vi "VIH Dialog - Project File Rules.vi"(6 "File set (All)":enum32{"ALL", "lost"}(ring), 11 "Project Tree":T1) -> (0 "OK out":bool, 2 "File Paths":path[](array[path]))   [LabVIEW 2014]
doc: "::: VI Helpeks :::\nCopyright (c) 2000-2026 Konstantin Shifershteyn. All rights reserved."
uses:
  VIH Project Tree Typedef - Tree Refnum.ctl
  _VIH HelpGen - Palette.llb/VIH HelpGen Typedef - Palette - Item Type Enum.ctl
  <vilib>/Utility/miscctls.llb/LVRowAndColumnUnsignedTypeDef.ctl
panel:
  in  "QualifiedNames":bool caption="Show qualified VI names"
  in  "KindOfFile":enum16{"All File Rules", "Lost Rules"}(ring) caption="Category Selector"
  in  "DirectSortColumn":i32
  in  "Files tmp":path[](array[path])
  in  "FileList":i32[](listbox) caption="Rule List"
  in  "%OK":bool
  out "Sel Path":path caption="File Path"
  in  "%Cancel":bool caption="Cloce"
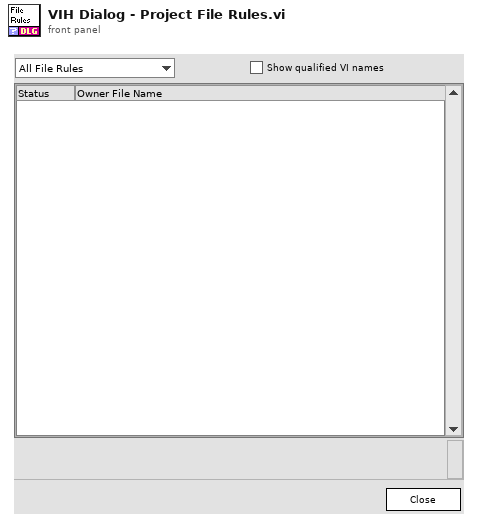
[diagram p1: front panel]
types:
  T1 = typedef "VIH Project Tree Typedef - Tree Refnum.ctl" = refnum<vi>
  T2 = typedef "VIH HelpGen Typedef - Palette - Item Type Enum.ctl" = enum32{"<Invalid>", "<unknown>", "VI", "Menu", "LV Func", "Express VI", "Poly VI", "CTL", "HTML"}
  T3 = cluster{"Types":T2[], "Item Paths":path[], "Lost Flags":bool[], "Names":string[]}
  T4 = enum8{"Enabled", "Disabled", "Disabled and Grayed Out"}
  T5 = enum16{"get", "get all", "set", "Init", "delete", "rename"}
  T6 = typedef "LVRowAndColumnUnsignedTypeDef.ctl" = cluster{"Row":u32, "Column":u32}
  T7 = typedef "LVPoint32TypeDef.ctl" = cluster{"Horizontal":i32, "Vertical":i32}
  T8 = typedef "LVRowAndColumnTypeDef.ctl" = cluster{"Row":i32, "Column":i32}
  T9 = typedef "lveventtype.ctl" = enum32{"Null", "Timeout", "Annotation Menu Selection", "Annotation Menu Selection?", "App Instance Close", "App Instance Close?", "Autoscale Range Change", "Bookmark Info Change", "Cell Edit", "Cell Edit?", "Cursor Grab", "Cursor Grab?", "Cursor Menu Selection", "Cursor Menu Selection?", "Cursor Move", "Cursor Release", "Data Change", "Direction Change", "Display State Change", "Drag Ended", "Drag Enter", "Drag Leave", "Drag Over", "Drag Source Update", "Drag Starting", "Drag Starting?", "Drop", "Exec State Change", "Key Down", "Key Down?", "Key Repeat", "Key Repeat?", "Key Up", "Listbox Double Click", "Menu Activation?", "Menu Selection (App)", "Menu Selection? (App)", "Menu Selection (User)", "Mouse Down", "Mouse Down?", "Mouse Enter", "Mouse Leave", "Mouse Move", "Mouse Up", "Mouse Wheel", "NI Security User Change (App)", "Pane Size", "Panel Close", "Panel Close?", "Panel Resize", "Plot Attribute Change", "Scale Range Change", "Shortcut Menu Activation?", "Shortcut Menu Selection (App)", "Shortcut Menu Selection? (App)", "Shortcut Menu Selection (User)", "Tree Double Click", "Tree Drag", "Tree Drag?", "Tree Drop", "Tree Drop?", "Tree Item Close", "Tree Item Close?", "Tree Item Open", "Tree Item Open?", "User Event", "Value Change"}
  T10 = cluster{"Item/File Type":T2, "Item ID out":path, bool}
  T11 = cluster{"Types":T2[], "Paths":path[], "Dynamic":enum16{"Dyn", "Stat", "Both"}[], "Can be built":bool[], "DynFileNotFound":bool[]}
  T12 = cluster{T2[], "Item Paths":path[], bool[], string[]}
  T13 = typedef "VIH HelpGen Typedef - Cluster - File Rule.ctl" = cluster{"OutName":string, "BuildHelp":T14, "Source Paths":T15, "Target Paths":T16, "DscrMode":T17, "Description":string, "Control Rules":T18[], "Flags":T20, "Ctl_DscrMode":T17, "Ctl_ClustMembers":T14, "Ctl_EnumValues":T14, "MenuItemIcons":T14, "%Comments":string, "DetailsMode":T17, "DetailsText":string, "ProductInfoMode":T14, "ProductInfoText":string}
  T14 = typedef "VIH HelpGen Typedef - Enum - Default,Enable,Disable.ctl" = enum16{"Default", "Enable", "Disable"}
  T15 = typedef "VIH HelpGen Typedef - Cluster - File Rule - Source Paths.ctl" = cluster{"CSS Files":path[], "JS Files":path[], "Html Template":path}
  T16 = typedef "VIH HelpGen Typedef - Cluster - File Rule - Target Paths.ctl" = cluster{"HTML Dir":path, "Image Dir":path, "CSS Dir":path, "JS Dir":path}
  T17 = typedef "VIH HelpGen Typedef - Enum - Description Mode.ctl" = enum16{"Default", "Description", "Description1", "Description2", "Custom", "None"}
  T18 = typedef "VIH HelpGen Typedef - Cluster - Control Rule.ctl" = cluster{"CtrlID":string, "CustomRule":bool, "DscrMode":T17, "Description":string, "ClusterMembers":T14, "EnumValues":T14, "EnumValDscr":T19[], "CustomName":string}
  T19 = typedef "VIH HelpGen Typedef - Cluster - Enum Value Info.ctl" = cluster{"Value":ext, "String":string, "Description":string}
  T20 = typedef "VIH HelpGen Typedef - Cluster - Group Rule - Flags.ctl" = cluster{"Override CSS Files":bool, "Override JS Files":bool, "Override Ctl Rules":bool}
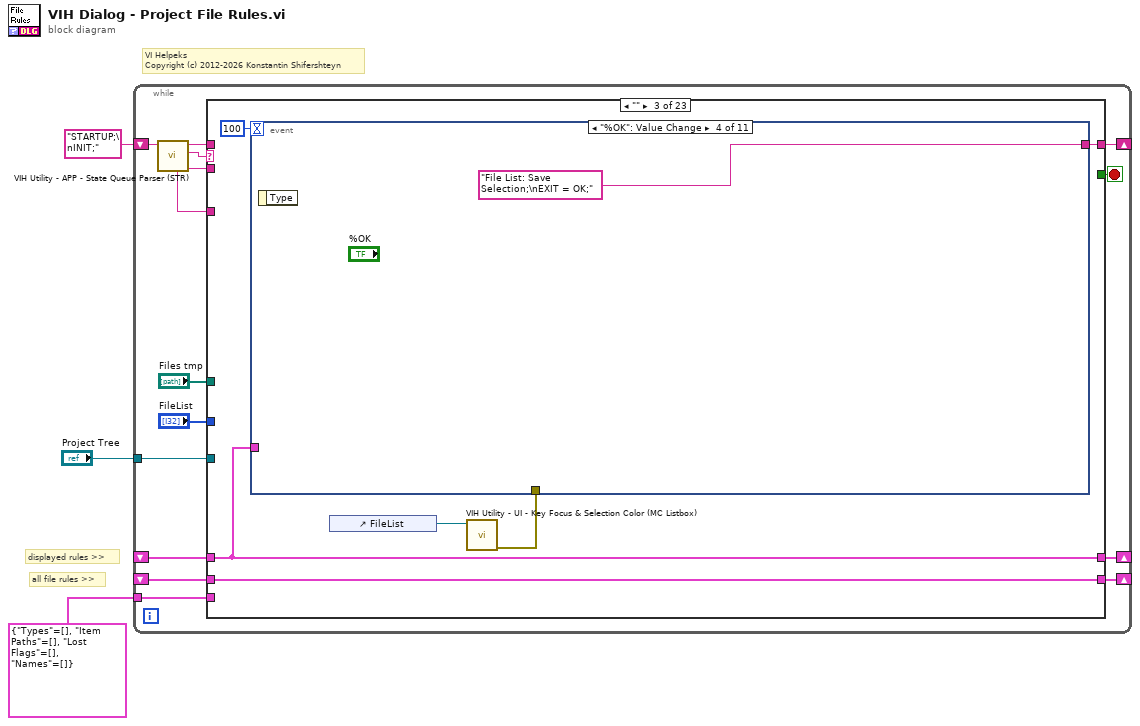
[diagram p0: block diagram]
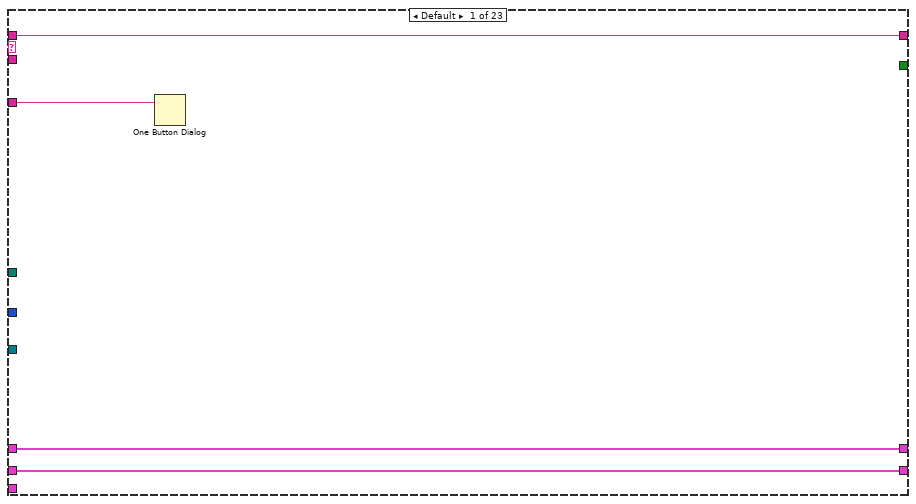
[diagram p2: hidden frame]
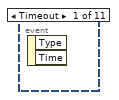
[diagram p4: hidden frame]
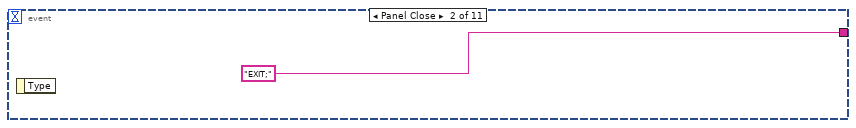
[diagram p5: hidden frame]
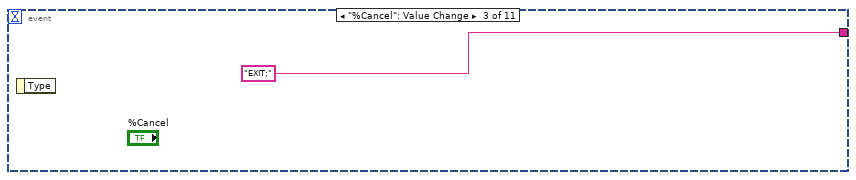
[diagram p6: hidden frame]
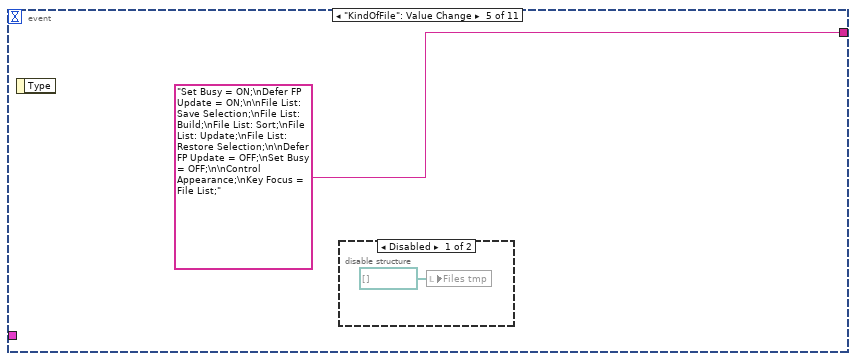
[diagram p7: hidden frame]
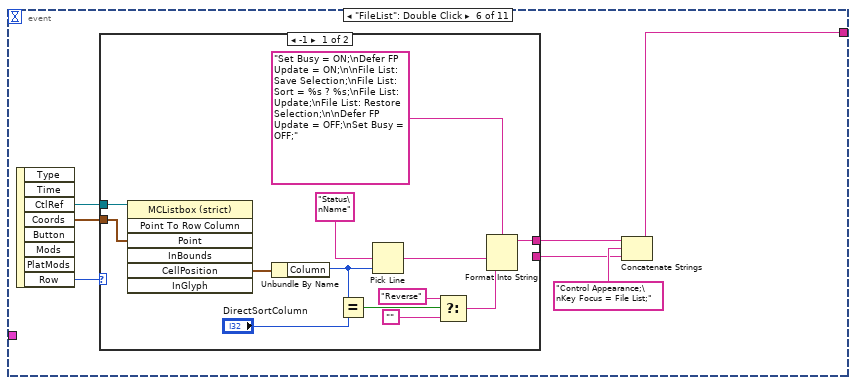
[diagram p9: hidden frame]
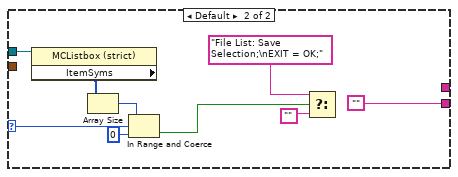
[diagram p10: hidden frame]
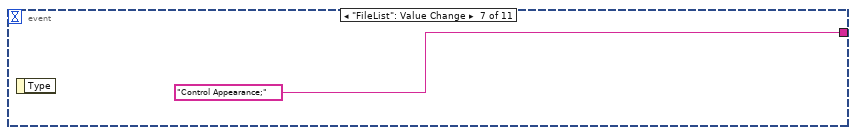
[diagram p11: hidden frame]
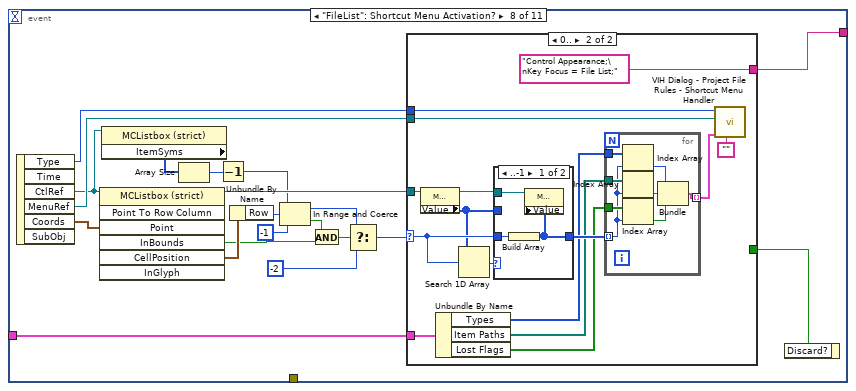
[diagram p12: hidden frame]
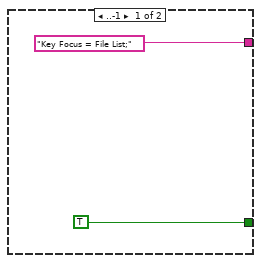
[diagram p13: hidden frame]
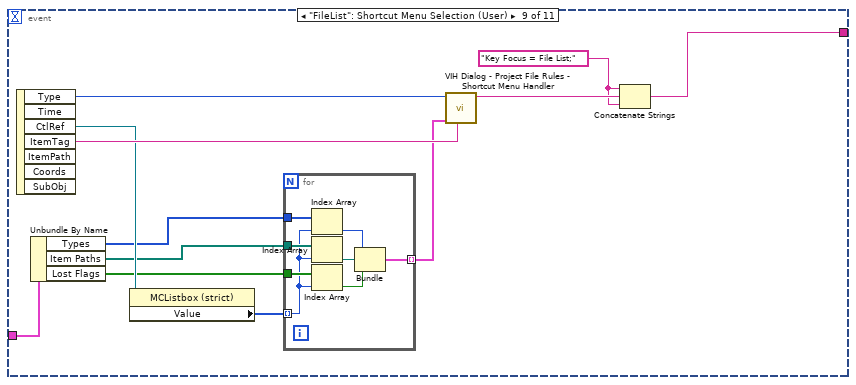
[diagram p15: hidden frame]
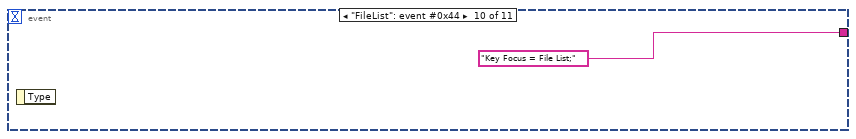
[diagram p16: hidden frame]
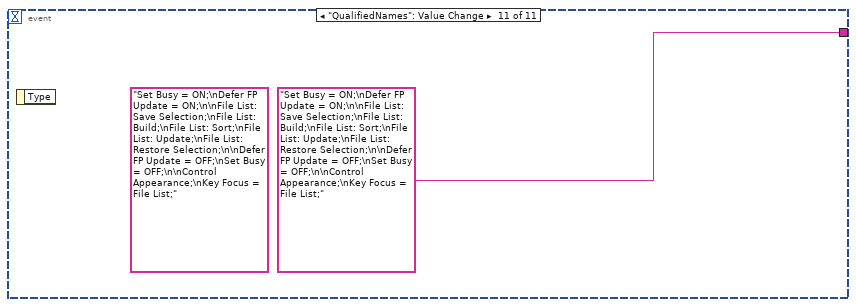
[diagram p17: hidden frame]
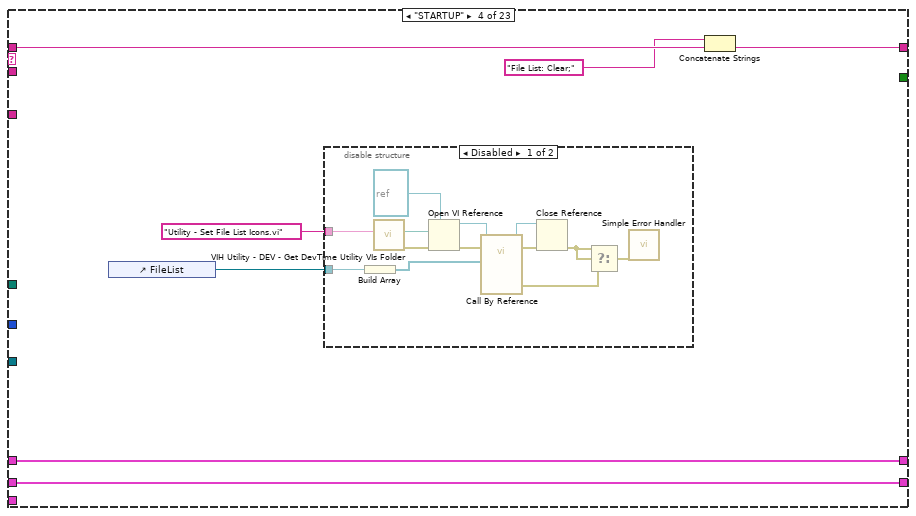
[diagram p18: hidden frame]
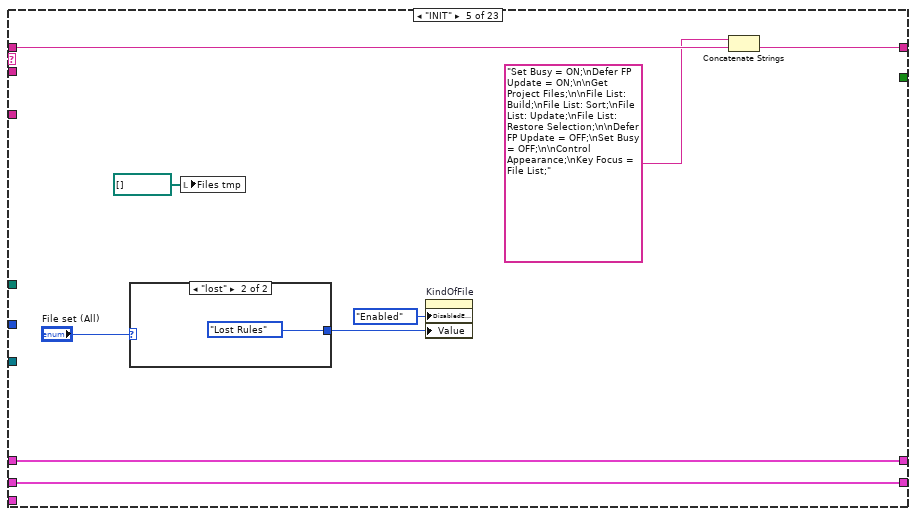
[diagram p20: hidden frame]
diagram:
  # "VI Helpeks\nCopyright (c) 2012-2026 Konstantin Shifershteyn"
  # "displayed rules >>"
  # "all file rules >>"
  n1 = while {
    shift-right: [w16] -> _
    shift-left: "STARTUP;\nINIT;" -> [w18]
    tunnel: "Project Tree" -> [w11]
    shift-right: [w10] -> _
    shift-left: _ -> [w9]
    shift-right: [w8] -> _
    shift-left: _ -> [w7]
    tunnel: T3 {"Types"=[], "Item Paths"=[], "Lost Flags"=[], "Names"=[]} ("output cluster") -> [w4]
    stop <- w13 stop-if-true
    n2 = call "VIH Utility - APP - State Queue Parser (STR).vi"("input queue"=w18) -> ("state parameters"=w12:string, "state"=w17:string, "remained queue"=w15:string, "complete state specifier"=w14:string)  [unwired: 5 in]
    n3 = case shown="\"\"" w17 {
      tunnel: [w22 w25 w30 w139 w165 "File List: Clear;\nHALT;" w189 w198 w202 w208 w213 w223 w232 w242 w269 w342 w417 w432 w451 w471 w475 w483 w517] -> w16
      tunnel: w15 -> [w22 w25 _ w142 w166 _ w189 w198 w202 w208 w213 w223 w232 w242 w269 w342 w417 w432 w451 w471 w475 w486 w520]
      tunnel: w14 -> [w21 _ _ _ _ _ _ _ _ _ _ _ _ _ _ _ _ _ _ _ _ _ _]
      tunnel: [_ _ _ _ _ _ TRUE _ _ _ _ _ _ _ _ _ _ _ _ _ _ _ _] -> w13
      tunnel: w12 -> [_ _ _ _ _ w174 _ _ w199 w203 w210 _ _ _ _ w331 _ _ _ _ _ w484 _]
      tunnel: w11 -> [_ _ _ _ _ _ _ _ _ _ _ _ _ w241 _ _ _ _ _ _ _ w481 _]
      tunnel: [w20 w24 w29 w144 w163 w172 w187 w196 w200 w206 w211 w222 w230 w237 w268 w343 w418 w433 w452 w472 w473 w477 w518] -> w10
      tunnel: w9 -> [w20 w24 w29 w144 w163 w172 _ w196 w200 w206 w211 w222 w230 _ w268 w343 w418 w433 w452 w472 w473 w477 w518]
      tunnel: [w19 w23 w28 w143 w162 w171 w187 w197 w201 w207 w212 w221 w231 w237 w261 w336 w416 w431 w450 w470 w474 w485 w519] -> w8
      tunnel: w7 -> [w19 w23 w28 w143 w162 w171 _ w197 w201 w207 w212 w221 w231 _ _ w341 w416 w431 w450 w470 w474 w485 w519]
      tunnel: "FileList" -> [_ _ _ _ _ w170 _ _ _ _ _ w220 _ _ _ _ _ w430 _ _ _ _ _]
      tunnel: "Files tmp" -> [_ _ _ _ _ _ _ _ _ _ _ _ _ _ _ _ _ _ w438 _ _ _ _]
      tunnel: w4 -> [_ _ _ _ _ _ w187 _ _ _ _ _ _ _ w257 w335 _ _ _ _ _ _ _]
      frame Default {
        n4 = One Button Dialog(message=w21) -> ()  [unwired: 1 in, 1 out]
      }
      frame "#" {
      }
      frame "" {
        n5 = control-ref of="FileList"() -> (w27:refnum<vi>)
        n6 = call "VIH Utility - UI - Key Focus & Selection Color (MC Listbox).vi"("MCListbox Refnum"=w27) -> ("error out"=w26:errorcluster)  [unwired: 8 in, 2 out]
        n7 = event shown="[3] \"%OK\": Value Change" {
          selector: _ -> [_ _ _ _ _ _ _ _ _ _ _]
          dyn-events: _ -> [_ _ _ _ _ _ _ _ _ _ _]
          timeout: 100 -> [_ _ _ _ _ _ _ _ _ _ _]
          tunnel: [_ "EXIT;" "EXIT;" "File List: Save Selection;\nEXIT = OK;" "Set Busy = ON;\nDefer FP Update = ON;\n\nFile List: Save Selection;\nFile List: Build;\nFile List: Sort;\nFile List: Update;\nFile List: Restore Selection;\n\nDefer FP Update = OFF;\nSet Busy = OFF;\n\nControl Appearance;\nKey Focus = File List;" w39 "Control Appearance;" w70 w120 "Key Focus = File List;" ("string") "Set Busy = ON;\nDefer FP Update = ON;\n\nFile List: Save Selection;\nFile List: Build;\nFile List: Sort;\nFile List: Update;\nFile List: Restore Selection;\n\nDefer FP Update = OFF;\nSet Busy = OFF;\n\nControl Appearance;\nKey Focus = File List;"] -> w30
          tunnel: w28 -> [_ _ _ _ _ _ _ w78 w122 _ _]
          tunnel: w26 -> [_ _ _ _ _ _ _ _ _ _ _]
          event Timeout {
            n8 = event-data() -> ()  [unwired: 1 in, 2 out]
          }
          event Panel Close {
            n9 = event-data() -> ()  [unwired: 1 in, 1 out]
          }
          event "%Cancel": Value Change {
            n10 = event-data() -> ()  [unwired: 1 in, 1 out]
          }
          event "%OK": Value Change {
            n11 = event-data() -> ()  [unwired: 1 in, 1 out]
          }
          event "KindOfFile": Value Change {
            n12 = event-data() -> ()  [unwired: 1 in, 1 out]
            n13 = disable-structure shown="Disabled" {
              frame Disabled {
                n14 = local write "Files tmp"(path[] [] ("Files tmp")) -> ()
              }
              frame Enabled {
              }
            }
          }
          event "FileList": Double Click {
            n15 = event-data() -> ("CtlRef"=w42:refnum<vi>, "Coords"=w41:T7, "Row"=w43:i32)  [unwired: 1 in, 5 out]
            n16 = case shown="-1" w43 {
              selector: w43 -> [_ w64]
              tunnel: w42 -> [w56 w65]
              tunnel: w41 -> [w55 _]
              tunnel: [w50 _] -> w40
              tunnel: [_ ""] -> w37
              frame -1 {
                n17 = invoke class="MCListbox (strict)" method="Point To Row Column"(reference=w56, "Point"=w55) -> ("CellPosition"=w54:T8)  [unwired: 5 in, 6 out]
                n18 = Unbundle By Name(w54) -> ("Column"=w49:i32)
                n19 = Equal?(x=w49, y="DirectSortColumn") -> (x = y?=w45:bool)
                n20 = Pick Line(multi-line string="Status\nName", line index=w49) -> (output string=w51:string)  [unwired: 1 in]
                n21 = Select(t="Reverse", s=w45, f="") -> (s? t:f=w44:string)
                n22 = Format Into String(format string="Set Busy = ON;\nDefer FP Update = ON;\n\nFile List: Save Selection;\nFile List: Sort = %s ? %s;\nFile List: Update;\nFile List: Restore Selection;\n\nDefer FP Update = OFF;\nSet Busy = OFF;", w51, w44) -> (resulting string=w50:string)  [unwired: 2 in, 1 out]
              }
              frame Default {
                n23 = property class="MCListbox (strict)"(reference=w65) -> ("ItemSyms"=w63:i32[])  [unwired: 1 in, 2 out]
                n24 = Array Size(array=w63) -> (size(s)=w62:i32)
                n25 = In Range and Coerce(upper limit=w62, x=w64, lower limit=0) -> (In Range?=w59:bool)  [unwired: 1 out]
                n26 = Select(t="File List: Save Selection;\nEXIT = OK;", s=w59, f="") -> ()  [unwired: 1 out]
              }
            }
            n27 = Concatenate Strings(w40, "Control Appearance;\nKey Focus = File List;", w37) -> (w39:string)
          }
          event "FileList": Value Change {
            n28 = event-data() -> ()  [unwired: 1 in, 1 out]
          }
          event "FileList": Shortcut Menu Activation? {
            n29 = event-data() -> ("Type"=w80:T9, "CtlRef"=w77:refnum<vi>, "MenuRef"=w79:refnum<k9>, "Coords"=w86:T7)  [unwired: 1 in, 2 out]
            n30 = invoke class="MCListbox (strict)" method="Point To Row Column"(reference=w77, "Point"=w86) -> (reference out=w81:refnum<vi>, "InBounds"=w69:bool, "CellPosition"=w85:T8)  [unwired: 5 in, 4 out]
            n31 = property class="MCListbox (strict)"(reference=w77) -> ("ItemSyms"=w75:i32[])  [unwired: 1 in, 2 out]
            n32 = Array Size(array=w75) -> (size(s)=w74:i32)
            n33 = Decrement(x=w74) -> (x-1=w73:i32)
            n34 = Unbundle By Name(w85) -> ("Row"=w76:i32)
            n35 = In Range and Coerce(upper limit=w73, x=w76, lower limit=-1) -> (coerced(x)=w71:i32, In Range?=w68:bool)
            n36 = And(x=w68, y=w69) -> (x .and. y?=w67:bool)
            n37 = Select(t=w71, s=w67, f=-2) -> (s? t:f=w83:i32)
            n38 = case shown="0.." w83 {
              selector: w83 -> [_ w100]
              tunnel: [TRUE _] -> w82
              tunnel: w81 -> [_ w103]
              tunnel: w80 -> [_ w99]
              tunnel: w79 -> [_ w98]
              tunnel: w78 -> [_ w93]
              tunnel: ["Key Focus = File List;" "Control Appearance;\nKey Focus = File List;"] -> w70
              frame ..-1 {
              }
              frame 0.. {
                n39 = property class="MCListbox (strict)"(reference=w103) -> (reference out=w102:refnum<vi>, "Value"=w96:i32[])  [unwired: 1 in, 1 out]
                n40 = Unbundle By Name(w93) -> ("Types"=w89:T2[], "Item Paths"=w90:path[], "Lost Flags"=w94:bool[])
                n41 = Search 1D Array(1D array=w96, element=w100) -> (index of element=w101:i32)  [unwired: 1 in]
                n42 = case shown="..-1" w101 {
                  tunnel: w102 -> [w114 _]
                  tunnel: w100 -> [w113 _]
                  tunnel: [w112 w115] -> w95
                  tunnel: w96 -> [_ w115]
                  frame ..-1 {
                    n43 = Build Array(w113) -> (w112:i32[])
                    n44 = property class="MCListbox (strict)"(reference=w114, "Value"=w112) -> ()  [unwired: 1 in, 2 out]
                  }
                  frame 0.. {
                  }
                }
                n45 = for {
                  tunnel: w95 -> [w106] mode=indexing
                  tunnel: w94 -> [w111]
                  tunnel: w90 -> [w110]
                  tunnel: [w107] -> w92 mode=indexing
                  tunnel: w89 -> [w105]
                  n46 = Index Array(array=w105, index=w106) -> (element=w104:T2)
                  n47 = Index Array(array=w110, index=w106) -> (element=w109:path)
                  n48 = Index Array(array=w111, index=w106) -> (element=w108:bool)
                  n49 = Bundle("Item/File Type"=w104, "Item ID out"=w109, w108) -> (w107:T10)  [unwired: 1 in]
                }
                n50 = call "VIH Dialog - Project File Rules - Shortcut Menu Handler.vi"("Menu Tag"="", "Files"=w92, "MenuRef"=w98, "Event Type"=w99) -> ()  [unwired: 7 in, 1 out]
              }
            }
            n51 = event-data("Discard?"=w82) -> ()  [unwired: 1 in, 1 out]
          }
          event "FileList": Shortcut Menu Selection (User) {
            w117 = "Key Focus = File List;" ("string")
            n52 = event-data() -> ("Type"=w127:T9, "CtlRef"=w124:refnum<vi>, "ItemTag"=w125:string)  [unwired: 1 in, 4 out]
            n53 = Unbundle By Name(w122) -> ("Types"=w116:T2[], "Item Paths"=w119:path[], "Lost Flags"=w121:bool[])
            n54 = property class="MCListbox (strict)"(reference=w124) -> ("Value"=w123:i32[])  [unwired: 1 in, 2 out]
            n55 = for {
              tunnel: w123 -> [w129] mode=indexing
              tunnel: w121 -> [w135]
              tunnel: w119 -> [w134]
              tunnel: [w131] -> w118 mode=indexing
              tunnel: w116 -> [w130]
              n56 = Index Array(array=w130, index=w129) -> (element=w128:T2)
              n57 = Index Array(array=w134, index=w129) -> (element=w133:path)
              n58 = Index Array(array=w135, index=w129) -> (element=w132:bool)
              n59 = Bundle("Item/File Type"=w128, "Item ID out"=w133, w132) -> (w131:T10)  [unwired: 1 in]
            }
            n60 = call "VIH Dialog - Project File Rules - Shortcut Menu Handler.vi"("Menu Tag"=w125, "Files"=w118, "Event Type"=w127) -> ("States spec"=w126:string)  [unwired: 8 in]
            n61 = Concatenate Strings(w117, w126, w117) -> (w120:string)
          }
          event "FileList": event #0x44 {
            n62 = event-data() -> ()  [unwired: 1 in, 1 out]
          }
          event "QualifiedNames": Value Change {
            (unwired) "Set Busy = ON;\nDefer FP Update = ON;\n\nFile List: Save Selection;\nFile List: Build;\nFile List: Sort;\nFile List: Update;\nFile List: Restore Selection;\n\nDefer FP Update = OFF;\nSet Busy = OFF;\n\nControl Appearance;\nKey Focus = File List;"
            n63 = event-data() -> ()  [unwired: 1 in, 1 out]
          }
        }
      }
      frame "STARTUP" {
        n64 = control-ref of="FileList"() -> (w141:refnum<vi>)
        n65 = disable-structure shown="Disabled" {
          disable-tunnel: w141 -> [w148 _]
          disable-tunnel: "Utility - Set File List Icons.vi" ("Utility VI Name") -> [w147 _]
          frame Disabled {
            n66 = Build Array(w148) -> (w146:refnum<vi>[])
            n67 = call "VIH Utility - DEV - Get DevTime Utility VIs Folder.vi"("Utility VI Name"=w147) -> ("error out"=w154:errorcluster, "Utility VIs Path"=w153:path)  [unwired: 8 in, 1 out]
            n68 = Open VI Reference(type specifier VI Refnum (for type only)=refnum<vi> refnum, vi path=w153, error in (no error)=w154) -> (vi reference=w156:refnum<vi>, error out=w157:errorcluster)  [unwired: 3 in]
            n69 = call-by-ref "?"(reference=w156, error in=w157, "MCListbox Refnums"=w146) -> (reference out=w151:refnum<vi>, error out=w152:errorcluster, 0:"error out"=w149:errorcluster)  [unwired: 10 in]
            n70 = Close Reference(reference=w151, error in (no error)=w152) -> (error out=w145:errorcluster)
            n71 = Select(t=w145, s=w145, f=w149) -> (s? t:f=w150:errorcluster)
            n72 = call <vilib>:"Simple Error Handler.vi"("error in (no error)"=w150) -> ()  [unwired: 4 in, 5 out]
          }
          frame Enabled {
          }
        }
        n73 = Concatenate Strings("File List: Clear;" ("string"), w142) -> (w139:string)
      }
      frame "INIT" {
        n74 = case shown="\"lost\"" "File set (All)" {
          tunnel: [enum16{"All File Rules", "Lost Rules"}."All File Rules" ("KindOfFile") enum16{"All File Rules", "Lost Rules"}."Lost Rules" ("KindOfFile")] -> w159
          frame "ALL" {
          }
          frame "lost" {
          }
        }
        n75 = local write "Files tmp"(path[] [] ("Files tmp")) -> ()
        n76 = property on="KindOfFile" class="Enum (strict)"("DisabledEnum"=T4."Enabled" ("Disabled"), "Value"=w159) -> ()  [unwired: 2 in, 2 out]
        n77 = Concatenate Strings("Set Busy = ON;\nDefer FP Update = ON;\n\nGet Project Files;\n\nFile List: Build;\nFile List: Sort;\nFile List: Update;\nFile List: Restore Selection;\n\nDefer FP Update = OFF;\nSet Busy = OFF;\n\nControl Appearance;\nKey Focus = File List;", w166) -> (w165:string)
      }
      frame "EXIT" {
        n78 = case shown="\"Find In Tree\"" w174 {
          tunnel: [_ TRUE TRUE] -> w173
          tunnel: w171 -> [_ _ w180]
          tunnel: w170 -> [_ _ w178]
          tunnel: [_ _ w177] -> w169
          frame Default {
          }
          frame "OK" {
          }
          frame "Find In Tree" {
            n79 = Unbundle By Name(w180) -> ("Item Paths"=w179:path[])
            n80 = for {
              tunnel: w179 -> [w184]
              tunnel: w178 -> [w183] mode=indexing
              tunnel: [w182] -> w177 mode=indexing
              n81 = Index Array(array=w184, index=w183) -> (element=w182:path)
            }
          }
        }
        "OK out" <- w173
        "File Paths" <- w169
      }
      frame "HALT" {
        n82 = Call Chain() -> (call chain=w185:string[])
        n83 = Array Size(array=w185) -> (size(s)=w186:i32)
        n84 = case shown="2.." w186 {
          frame ..1 {
          }
          frame 2.. {
            n85 = for {
              N: 100 -> [_]
              tunnel: [w193] -> w190
              stop <- w193 continue-if-true
              n86 = property class="VI"("Front Panel.Open"=FALSE ("Front Panel Window:Open")) -> ("Front Panel.Open"=w193:bool)  [unwired: 2 in, 2 out]
              n87 = Wait (ms)(milliseconds to wait=u32 10) -> ()  [unwired: 1 out]
            }
            n88 = stacked-sequence {
              tunnel: w190 -> [_]
              frame #0 {
                n89 = property on="KindOfFile" class="Enum (strict)"("DisabledEnum"=T4."Enabled" ("Disabled")) -> ()  [unwired: 2 in, 2 out]
              }
            }
          }
        }
      }
      frame "--------------------------- 1" {
      }
      frame "Set Busy" {
        n90 = case shown="\"ON\"" w199 {
          frame "OFF", Default {
            n91 = call <vilib>:"Unset Busy.vi"() -> ()  [unwired: 11 in, 1 out]
          }
          frame "ON" {
            n92 = call <vilib>:"Set Busy.vi"() -> ()  [unwired: 10 in, 2 out]
          }
        }
      }
      frame "Defer FP Update" {
        n93 = case shown="\"ON\"" w203 {
          tunnel: [_ TRUE] -> w205
          frame "OFF", Default {
          }
          frame "ON" {
          }
        }
        n94 = property class="VI"() -> ("Front Panel"=w204:refnum<vi>)  [unwired: 2 in, 2 out]
        n95 = property class="Pnl"(reference=w204, "Defer Panel Updates"=w205) -> ()  [unwired: 1 in, 2 out]
      }
      frame "Key Focus" {
        n96 = case shown="\"File List\"" w210 {
          frame Default {
          }
          frame "File List" {
            n97 = control-ref of="FileList"() -> (w215:refnum<vi>)
            n98 = call "VIH Utility - UI - Key Focus & Selection Color (MC Listbox).vi"("F:Test/T:Set Key Focus (F)"=TRUE, "MCListbox Refnum"=w215) -> ()  [unwired: 7 in, 3 out]
          }
        }
      }
      frame "Control Appearance" {
        n99 = Array Size(array=w220) -> (size(s)=w218:i32)
        n100 = case shown="1" w218 {
          tunnel: w221 -> [_ w229]
          tunnel: w220 -> [_ w228]
          tunnel: [_ w226] -> w219
          tunnel: [_ TRUE] -> _
          frame Default {
          }
          frame 1 {
            n101 = Unbundle(w229) -> ("Item Paths"=w224:path[])  [unwired: 3 out]
            n102 = Index Array(array=w228) -> (element=w227:i32)  [unwired: 1 in]
            n103 = Index Array(array=w224, index=w227) -> (element=w226:path)
          }
        }
        "Sel Path" <- w219
        n104 = call "VIH Utility - UI - Boolean to Control Disable Status.vi"("Status in"=FALSE) -> ("Control Disable if False"=w217:u8)  [unwired: 3 in, 1 out]
        n105 = property on="%OK" class="Bool"("DisabledEnum"=w217) -> ()  [unwired: 2 in, 2 out]
      }
      frame "--------------------------- 2" {
      }
      frame "Get Project Files" {
        n106 = call "VIH Project Tree - Get Project Files & Groups (Ext).vi"("Project Tree"=w241) -> ("Project Files"=w235:T11)  [unwired: 7 in, 3 out]
        n107 = Unbundle By Name(w235) -> ("Paths"=w240:path[])
        n108 = call "VIH Project - Container - Item Rules.vi"("cmd (get)"=T5."get all") -> ("Item Paths"=w239:path[])  [unwired: 6 in, 4 out]
        n109 = for {
          tunnel: w240 -> [w248]
          tunnel: w239 -> [w244] mode=indexing
          tunnel: [w246] -> w238 mode=indexing
          tunnel: [w245] -> w234 mode=indexing
          tunnel: [w243] -> w233 mode=indexing
          n110 = call "VIH HelpGen - FILE - Get Type.vi"("File Path"=w244) -> ("File Type"=w245:T2)  [unwired: 8 in, 2 out]
          n111 = Search 1D Array(1D array=w248, element=w244) -> (index of element=w247:i32)  [unwired: 1 in]
          n112 = Strip Path(path=w244) -> (name=w243:string)  [unwired: 1 out]
          n113 = Less Than 0?(x=w247) -> (x < 0?=w246:bool)
        }
        n114 = Bundle(w234, "Item Paths"=w239, w238, w233) -> (w237:T12)  [unwired: 1 in]
      }
      frame "File List: Build" {
        n115 = Unbundle(w268) -> ("Types"=w258:T2[], "Item Paths"=w267:path[], "Lost Flags"=w256:bool[], "Names"=w253:string[])
        n116 = Array Size(array=w258) -> (size(s)=w259:i32)
        n117 = for {
          N: w259 -> [_]
          shift-right: [w286] -> w265
          shift-left: w258 -> [w287]
          shift-right: [w285] -> w264
          shift-left: w267 -> [w281]
          shift-right: [w284] -> w251
          shift-left: 0 -> [w283]
          tunnel: "KindOfFile" -> [w282]
          shift-right: [w279] -> w255
          shift-left: w256 -> [w278]
          shift-right: [w274] -> w252
          shift-left: w253 -> [w275]
          tunnel: "QualifiedNames" -> [w270]
          i -> [w277]
          n118 = Index Array(array=w287, index=w277) -> (element=w273:T2)
          n119 = Index Array(array=w281, index=w277) -> (element=w280:path)
          n120 = Index Array(array=w278, index=w277) -> (element=w276:bool)
          n121 = case shown="\"VI\"" w273 {
            tunnel: [_ _ TRUE _ _ TRUE TRUE TRUE _] -> w272
            frame "<Invalid>" {
            }
            frame "<unknown>" {
            }
            frame "VI" {
            }
            frame "Menu" {
            }
            frame "LV Func" {
            }
            frame "Express VI" {
            }
            frame "Poly VI" {
            }
            frame "CTL" {
            }
            frame "HTML" {
            }
          }
          n122 = case shown="\"All File Rules\"" w282 {
            tunnel: [TRUE w318] -> w288
            tunnel: w276 -> [_ w318]
            frame "All File Rules" {
            }
            frame "Lost Rules" {
            }
          }
          n123 = And(x=w272, y=w270) -> (x .and. y?=w271:bool)
          n124 = case shown="True" w288 {
            tunnel: w287 -> [w297 w311]
            tunnel: [w297 w310] -> w286
            tunnel: [w296 w312] -> w285
            tunnel: w281 -> [w296 w307]
            tunnel: [w295 w309] -> w284
            tunnel: w283 -> [w295 w301]
            tunnel: w273 -> [_ w308]
            tunnel: w280 -> [_ w299]
            tunnel: [w294 w305] -> w279
            tunnel: w278 -> [w294 w306]
            tunnel: w276 -> [_ w304]
            tunnel: w275 -> [w293 w303]
            tunnel: [w293 w302] -> w274
            tunnel: w271 -> [_ w298]
            frame False {
            }
            frame True {
              n125 = case shown="False" w298 {
                tunnel: w299 -> [w314 w316]
                tunnel: [w313 w315] -> w300
                frame False {
                  n126 = Strip Path(path=w314) -> (name=w313:string)  [unwired: 1 out]
                }
                frame True {
                  n127 = call "VIH HelpGen - FILE - Get Qualified Filename.vi"("File Path"=w316) -> ("Qualified name"=w315:string)  [unwired: 9 in, 1 out]
                }
              }
              n128 = Replace Array Subset(array=w306, new element=w304, index=w301) -> (w305:bool[])
              n129 = Replace Array Subset(array=w311, new element=w308, index=w301) -> (w310:T2[])
              n130 = Replace Array Subset(array=w307, new element=w299, index=w301) -> (w312:path[])
              n131 = Increment(x=w301) -> (x+1=w309:i32)
              n132 = Replace Array Subset(array=w303, new element=w300, index=w301) -> (w302:string[])
            }
          }
        }
        n133 = Reshape Array(w265, w251) -> (w263:T2[])
        n134 = Reshape Array(w255, w251) -> (w254:bool[])
        n135 = Reshape Array(w264, w251) -> (w262:path[])
        n136 = Reshape Array(w252, w251) -> (w250:string[])
        n137 = Bundle(cluster=w257, "Types"=w263, "Item Paths"=w262, "Lost Flags"=w254, "Names"=w250) -> (w261:T3)
      }
      frame "File List: Sort" {
        n138 = Unbundle(w341) -> ("Types"=w340:T2[], "Item Paths"=w339:path[], "Lost Flags"=w324:bool[], "Names"=w321:string[])
        n139 = Match Pattern(string=w331, regular expression="\\?") -> (before substring=w333:string, after substring=w334:string)  [unwired: 1 in, 2 out]
        n140 = call <vilib>:"Trim Whitespace.vi"("string"=w333) -> ("trimmed string"=w330:string)  [unwired: 1 in]
        n141 = call <vilib>:"Trim Whitespace.vi"("string"=w334) -> ("trimmed string"=w327:string)  [unwired: 1 in]
        n142 = case shown="\"Status\"" w330 {
          tunnel: w340 -> [w364 w392]
          tunnel: w339 -> [w362 w390]
          tunnel: [w366 w394] -> w338
          tunnel: [w365 w393] -> w337
          tunnel: [0 1] -> w325
          tunnel: w324 -> [w361 w389]
          tunnel: [w360 w388] -> w322
          tunnel: w321 -> [w359 w387]
          tunnel: [w358 w386] -> w319
          frame "Status" {
            n143 = for {
              tunnel: w362 -> [w385] mode=indexing
              tunnel: [w382] -> w368 mode=indexing
              tunnel: w361 -> [w381] mode=indexing
              tunnel: w359 -> [w379] mode=indexing
              i -> [w384]
              n144 = Not(x=w381) -> (.not. x?=w380:bool)
              n145 = To Lower Case(string=w379) -> (all lower case string=w383:string)
              n146 = Bundle(w380, w383, "Item ID out"=w385, w384) -> (w382:cluster{bool, string, "Item ID out":path, i32})  [unwired: 1 in]
            }
            n147 = Sort 1D Array(array=w368) -> (sorted array=w367:cluster{bool, string, "Item ID out":path, i32}[])
            n148 = for {
              tunnel: w367 -> [w378] mode=indexing
              tunnel: w364 -> [w377]
              tunnel: w362 -> [w376]
              tunnel: [w375] -> w366 mode=indexing
              tunnel: [w374] -> w365 mode=indexing
              tunnel: w361 -> [w373]
              tunnel: [w372] -> w360 mode=indexing
              tunnel: w359 -> [w371]
              tunnel: [w370] -> w358 mode=indexing
              n149 = Unbundle(w378) -> (w369:i32)  [unwired: 3 out]
              n150 = Index Array(array=w377, index=w369) -> (element=w375:T2)
              n151 = Index Array(array=w376, index=w369) -> (element=w374:path)
              n152 = Index Array(array=w373, index=w369) -> (element=w372:bool)
              n153 = Index Array(array=w371, index=w369) -> (element=w370:string)
            }
          }
          frame "Name", Default {
            n154 = for {
              tunnel: w390 -> [w411] mode=indexing
              tunnel: [w408] -> w396 mode=indexing
              tunnel: w387 -> [w407] mode=indexing
              i -> [w410]
              n155 = To Lower Case(string=w407) -> (all lower case string=w409:string)
              n156 = Bundle(w409, "Item ID out"=w411, w410) -> (w408:cluster{string, "Item ID out":path, i32})  [unwired: 1 in]
            }
            n157 = Sort 1D Array(array=w396) -> (sorted array=w395:cluster{string, "Item ID out":path, i32}[])
            n158 = for {
              tunnel: w395 -> [w406] mode=indexing
              tunnel: w392 -> [w405]
              tunnel: w390 -> [w404]
              tunnel: [w403] -> w394 mode=indexing
              tunnel: [w402] -> w393 mode=indexing
              tunnel: w389 -> [w401]
              tunnel: [w400] -> w388 mode=indexing
              tunnel: w387 -> [w399]
              tunnel: [w397] -> w386 mode=indexing
              n159 = Unbundle(w406) -> (w398:i32)  [unwired: 2 out]
              n160 = Index Array(array=w405, index=w398) -> (element=w403:T2)
              n161 = Index Array(array=w404, index=w398) -> (element=w402:path)
              n162 = Index Array(array=w401, index=w398) -> (element=w400:bool)
              n163 = Index Array(array=w399, index=w398) -> (element=w397:string)
            }
          }
        }
        n164 = case shown="\"Reverse\"" w327 {
          tunnel: w338 -> [w348 w357]
          tunnel: w337 -> [w347 w356]
          tunnel: [w348 w355] -> w329
          tunnel: [w347 w354] -> w328
          tunnel: [w346 -1] -> w326
          tunnel: w325 -> [w346 _]
          tunnel: [w345 w351] -> w323
          tunnel: w322 -> [w345 w352]
          tunnel: [w344 w349] -> w320
          tunnel: w319 -> [w344 w350]
          frame Default {
          }
          frame "Reverse" {
            n165 = Reverse 1D Array(array=w357) -> (reversed array=w355:T2[])
            n166 = Reverse 1D Array(array=w356) -> (reversed array=w354:path[])
            n167 = Reverse 1D Array(array=w352) -> (reversed array=w351:bool[])
            n168 = Reverse 1D Array(array=w350) -> (reversed array=w349:string[])
          }
        }
        n169 = local write "DirectSortColumn"(w326) -> ()
        n170 = Bundle(cluster=w335, "Types"=w329, "Item Paths"=w328, "Lost Flags"=w323, "Names"=w320) -> (w336:T3)
      }
      frame "File List: Update" {
        n171 = Unbundle(w416) -> ("Lost Flags"=w413:bool[], "Names"=w412:string[])  [unwired: 2 out]
        n172 = for {
          tunnel: [w422] -> w414 mode=indexing
          tunnel: w413 -> [w423] mode=indexing
          tunnel: [w427] -> w415 mode=indexing
          tunnel: w412 -> [w419] mode=indexing
          (unwired) "Linked" ("f")
          n173 = Select(t="Lost", s=w423, f="Ok") -> (s? t:f=w424:string)
          n174 = Select(t=3, s=w423, f=1) -> (s? t:f=w422:i32)
          n175 = Build Array(w424, w419) -> (w427:string[])
        }
        n176 = property on="FileList" class="MCListbox (strict)"("ItemNames"=w415, "ItemSyms"=w414) -> ()  [unwired: 2 in, 2 out]
      }
      frame "File List: Save Selection" {
        n177 = Unbundle(w431) -> ("Item Paths"=w428:path[])  [unwired: 3 out]
        n178 = for {
          tunnel: w430 -> [w436] mode=indexing
          tunnel: w428 -> [w435]
          tunnel: [w434] -> w429 mode=indexing
          n179 = Index Array(array=w435, index=w436) -> (element=w434:path)
        }
        n180 = local write "Files tmp"(w429) -> ()
      }
      frame "File List: Restore Selection" {
        n181 = Unbundle(w450) -> ("Item Paths"=w437:path[])  [unwired: 3 out]
        n182 = Array Size(array=w438) -> (size(s)=w448:i32)
        n183 = Initialize Array(0, w448) -> (w447:i32[])
        n184 = for {
          tunnel: w437 -> [w459]
          tunnel: w438 -> [w458] mode=indexing
          shift-right: [w456] -> w445
          shift-left: w447 -> [w455]
          shift-right: [w454] -> w444
          shift-left: 0 -> [w453]
          n185 = Search 1D Array(1D array=w459, element=w458) -> (index of element=w457:i32)  [unwired: 1 in]
          n186 = case shown="0.." w457 {
            selector: w457 -> [_ w465]
            tunnel: [w461 w462] -> w456
            tunnel: w455 -> [w461 w466]
            tunnel: [w460 w463] -> w454
            tunnel: w453 -> [w460 w464]
            frame ..-1 {
            }
            frame 0.. {
              n187 = Replace Array Subset(array=w466, new element=w465, index=w464) -> (w462:i32[])
              n188 = Increment(x=w464) -> (x+1=w463:i32)
            }
          }
        }
        n189 = Reshape Array(w445, w444) -> (w443:i32[])
        n190 = Sort 1D Array(array=w443) -> (sorted array=w440:i32[])
        n191 = control-ref of="FileList"() -> (w442:refnum<vi>)
        n192 = property on="FileList" class="MCListbox (strict)"("Value"=w440) -> (error out=w441:errorcluster)  [unwired: 2 in, 1 out]
        n193 = Index Array(array=w440) -> (element=w439:i32)  [unwired: 1 in]
        n194 = call "VIH Utility - UI - Make Row Visible (MC Listbox).vi"("error in"=w441, "Row"=w439, "MC Listbox Refnum"=w442) -> ()  [unwired: 7 in, 2 out]
      }
      frame "File List: Clear" {
        w467 = i32[] [] ("Item Symbols")
        n195 = property on="FileList" class="MCListbox (strict)"("TopLeft"=T6 {"Row"=0, "Column"=0} ("Top Left Visible Cell"), "Value"=w467, "ItemNames"=string[][] [] ("Item Names"), "ItemSyms"=w467) -> ()  [unwired: 2 in, 2 out]
      }
      frame "--------------------------- 3" {
      }
      frame "Rule: Find Target" {
        n196 = String To Path(string=w484) -> (path=w478:path)
        n197 = call "VIH Dialog - Project File List.vi"("Project Tree"=w481) -> ("OK out"=w479:bool, "File Path"=w480:path)  [unwired: 8 in, 1 out]
        n198 = Unbundle(w477) -> ("Item Paths"=w476:path[])  [unwired: 3 out]
        n199 = case shown="True" w479 {
          tunnel: [_ w503] -> w482
          tunnel: w480 -> [_ w501]
          tunnel: w478 -> [_ w500]
          tunnel: w476 -> [_ w502]
          frame False {
          }
          frame True {
            n200 = Strip Path(path=w500) -> (name=w499:string)  [unwired: 1 out]
            n201 = Strip Path(path=w501) -> (name=w498:string)  [unwired: 1 out]
            n202 = Search 1D Array(1D array=w502, element=w501) -> (index of element=w495:i32)  [unwired: 1 in]
            n203 = To Lower Case(string=w499) -> (all lower case string=w497:string)
            n204 = To Lower Case(string=w498) -> (all lower case string=w496:string)
            n205 = Greater Or Equal To 0?(x=w495) -> (x >= 0?=w493:bool)
            n206 = Not Equal?(x=w497, y=w496) -> (x != y?=w494:bool)
            n207 = Build Array(w493, w494) -> (w492:bool[])
            n208 = Search 1D Array(1D array=w492, element=TRUE) -> (index of element=w490:i32)  [unwired: 1 in]
            n209 = case shown="1" w490 {
              tunnel: [TRUE _ w507] -> w489
              tunnel: "ERROR:\nThe file you selected already has a rule linked." -> [_ w505 _]
              tunnel: "WARNING:\nThe file you selected has different name.\n\nAre you sure?" -> [_ _ w506]
              frame Default {
              }
              frame 0 {
                n210 = One Button Dialog(message=w505) -> ()  [unwired: 1 in, 1 out]
              }
              frame 1 {
                n211 = Two Button Dialog(message=w506) -> (T button?=w507:bool)  [unwired: 2 in]
              }
            }
            n212 = case shown="True" w489 {
              tunnel: [_ "Set Busy = ON;\nDefer FP Update = ON;\n\nGet Project Files;\n\nFile List: Build;\nFile List: Sort;\nFile List: Update;\nFile List: Restore Selection;\n\nDefer FP Update = OFF;\nSet Busy = OFF;\n\nControl Appearance;\nKey Focus = File List;"] -> w503
              tunnel: w500 -> [_ w509]
              tunnel: w501 -> [_ w508]
              frame False {
              }
              frame True {
                n213 = call "VIH Project - Container - Item Rules.vi"("Item Path"=w509) -> ("Item Rule out"=w510:T13, "Item Idx out"=w511:i32)  [unwired: 6 in, 3 out]
                n214 = Build Array(w508) -> (w514:path[])
                n215 = call "VIH Project - Container - Item Rules.vi"("cmd (get)"=T5."rename", "Item Rule"=w510, "Item Idx (-1)"=w511, "Item Path"=w508) -> ()  [unwired: 3 in, 5 out]
                n216 = local write "Files tmp"(w514) -> ()
              }
            }
          }
        }
        n217 = Concatenate Strings(w482, w486) -> (w483:string)
      }
      frame "Rule: Deleted" {
        n218 = local write "Files tmp"(path[] [] ("Files tmp")) -> ()
        n219 = Concatenate Strings("Set Busy = ON;\nDefer FP Update = ON;\n\nGet Project Files;\n\nFile List: Build;\nFile List: Sort;\nFile List: Update;\nFile List: Restore Selection;\n\nDefer FP Update = OFF;\nSet Busy = OFF;\n\nControl Appearance;\nKey Focus = File List;", w520) -> (w517:string)
      }
    }
  }
